vi "Main.vi"() -> ()   [LabVIEW 2018]
uses:
  Kompress.lvlib
panel:
  out "Decompressed String Size":i32
  out "Decompressed String":string
  out "Compressed String Size":i32
  out "Compressed String":string
  out "Input String Size":i32
  in  "Input String":string="p8ghobQyKtjzUzIhKCzvBaKCKBmhtb7283ARgSrl9PkbJoRdwPc1dwcj8u2oFV2nUiBOAn78Ad2IIrjzTtQyZJXJxGwasWFevUjShUP2e3znHiwX74VNoJgETWAH86R3YyvBQNR3MYMu21Tg9ifWKzXBhxgcm5BQdENaBFoRio95rfYKTwEFqfLsYR1Be9K6ABYgY5G1wNP9ZT35DnOAUj1Ywmuay0cbuQy44DAALULUFwE0hAsOyRikenUy4hss0K9sqBUFSYWpaBTFsZRj4sBxKuIX7GH3yeEj0FSkQeKBZiycZlmar4BMDkX5i5I1WzkvzTuQhAGnZFa7CHWz1POiln5OaTQHLcMA3jIFRSuAePc7ZOQkj255D1mEZgVjD18hRrb24wE1TOAJ2FIYFvQ4ZeAaDVQ1LU53PsKB98qWEz7aMPzk8v6etkvAEUdq42LXuQGm2pLeg0u9ufDCGeGWfxFtwV94uWnDrJmLwuK6fX1NR5YfCgbJo9MR3PjfMvoYqn45Ca5vjiaMpmm4yVD1jXGp3w3RlWYg10vOrcfW4zkPCBeElt9dpAhw5BS741OQFFWxrxbNzpLGxXOVDBCb..."
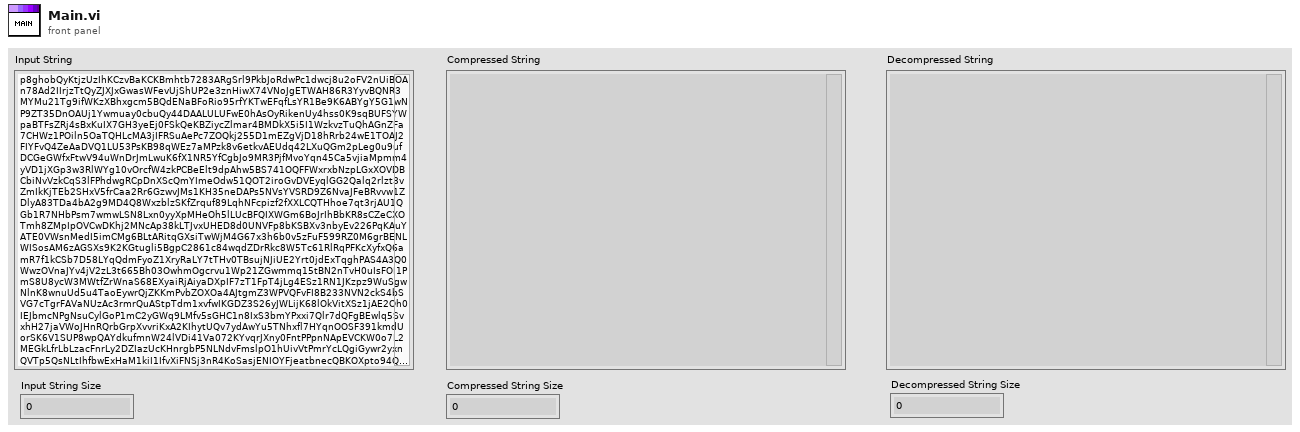
[diagram p1: front panel]
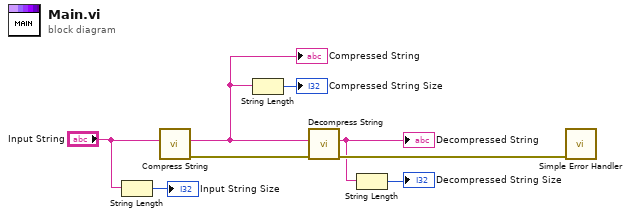
[diagram p0: block diagram]
diagram:
  n1 = String Length(string="Input String") -> (length=→"Input String Size":i32)
  n2 = call "Compress String.vi"("String"="Input String") -> ("error out"=w7:errorcluster, "Compressed String"=w4:string)  [unwired: 9 in]
  "Compressed String" <- w4
  n3 = String Length(string=w4) -> (length=→"Compressed String Size":i32)
  n4 = call "Decompress String.vi"("error in (no error)"=w7, "Compressed String"=w4) -> ("error out"=w6:errorcluster, "Decompressed String"=w2:string)  [unwired: 8 in]
  "Decompressed String" <- w2
  n5 = String Length(string=w2) -> (length=→"Decompressed String Size":i32)
  n6 = call <vilib>:"Simple Error Handler.vi"("error in (no error)"=w6) -> ()  [unwired: 4 in, 5 out]
